vi "Replace String in File.vi"(7 "File Path":path, 8 "error in":errorcluster, 9 "Replace String":string, 10 "Search String":string, 11 "IFile Manager in":refnum<class "IFile Manager.lvclass">) -> (0 "error out":errorcluster, 3 "IFile Manager out":refnum<class "IFile Manager.lvclass">)   [LabVIEW 2026, in "IFile Manager.lvclass"]
doc: "This VI replaces all instances of the search string by the replace strin in the provided text file."
uses:
  IFile Manager.lvclass
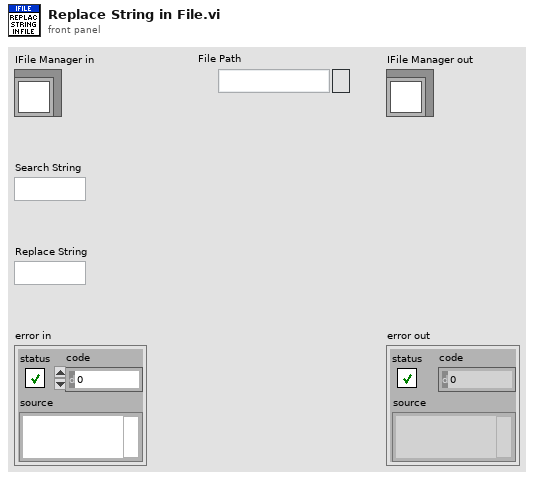
[diagram p1: front panel]
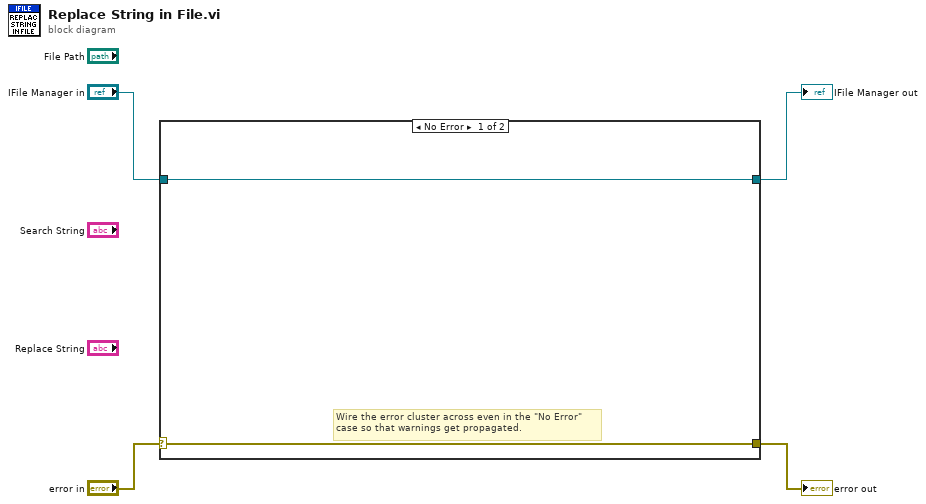
[diagram p0: block diagram]
diagram:
  n1 = case shown="No Error" "error in" {
    selector: "error in" -> [w6 w8]
    tunnel: [w6 w8] -> w3
    tunnel: [w5 w7] -> w1
    tunnel: "IFile Manager in" -> [w5 w7]
    frame No Error {
      # "Wire the error cluster across even in the \"No Error\"\ncase so that warnings get propagated."
    }
    frame Error {
    }
  }
  "error out" <- w3
  "IFile Manager out" <- w1
